vi "Test Create Instrument SMO.vi"(8 "error in (no error)":errorcluster) -> (0 "error out":errorcluster)   [LabVIEW 2019]
uses:
  <vilib>/addons/_JKI Toolkits/Caraya/classes/Assert/Assert Not Error.vi
  <vilib>/addons/_JKI Toolkits/Caraya/classes/Assert/Assert.lvclass
  <vilib>/addons/_JKI Toolkits/Caraya/classes/Test/Test.lvclass
  lvsrc/Framework-Template/SMOs/Instrument.Framework-Template/Instrument.Framework-Template.lvclass
panel:
  # "1. Run This VI\n\n2. SMOs will start in \"debug\" mode.\n  --> Stop the Test Launcher that opens\n\n3. SMOs will run in normal mode.\n  --> Stop the Test Launcher that opens."
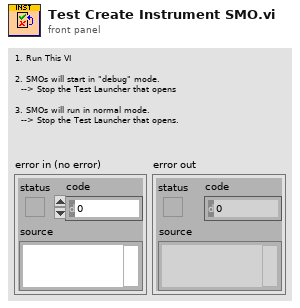
[diagram p1: front panel]
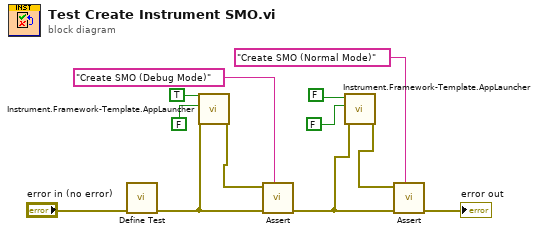
[diagram p0: block diagram]
diagram:
  n1 = call <vilib>:"Define Test.vi"("error in (no error)"="error in (no error)") -> ("error out"=w8:errorcluster)  [unwired: 9 in, 1 out]
  n2 = call "Instrument.Framework-Template.AppLauncher.vi"("error in"=w8, "Config Window"=FALSE ("Configuration Window? [T]"), "Debug Mode"=TRUE ("Debug Mode?")) -> ("error out"=w5:errorcluster)  [unwired: 8 in]
  n3 = call-poly <vilib>:"Assert.vi"("Label"="Create SMO (Debug Mode)", "error in (no error)"=w8, "Not Error?"=w5) -> ("error out"=w2:errorcluster)  [unwired: 7 in, 1 out]
  n4 = call "Instrument.Framework-Template.AppLauncher.vi"("error in"=w2, "Config Window"=FALSE ("Configuration Window? [T]"), "Debug Mode"=FALSE ("Debug Mode?")) -> ("error out"=w1:errorcluster)  [unwired: 8 in]
  n5 = call-poly <vilib>:"Assert.vi"("Label"="Create SMO (Normal Mode)", "error in (no error)"=w2, "Not Error?"=w1) -> ("error out"=→"error out":errorcluster)  [unwired: 7 in, 1 out]
